vi "Numerique_vers_chaine.vi"(0 "Valeur numérique":dbl) -> (1 "Chaine sans zéros inutiles":string, 2 "Chaîne brute":string)   [LabVIEW 2022 SP3]
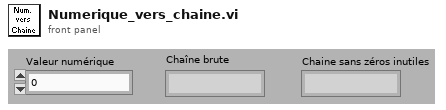
[diagram p1: front panel]
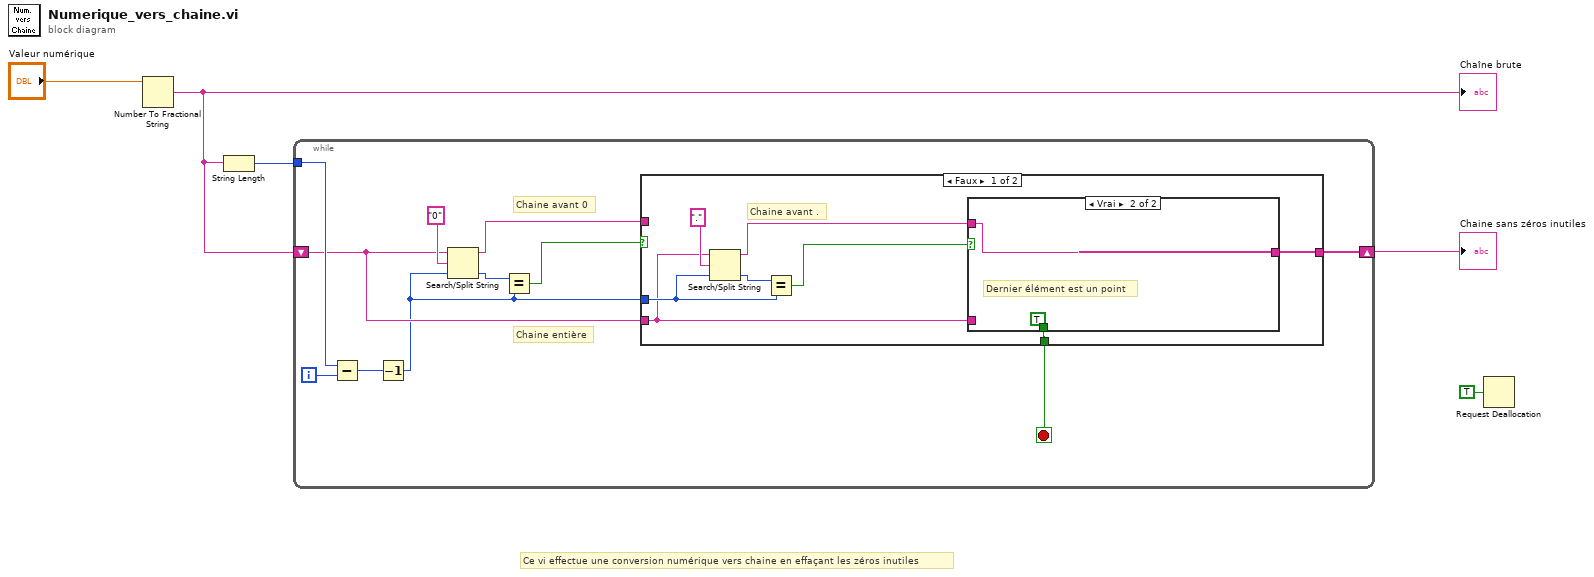
[diagram p0: block diagram]
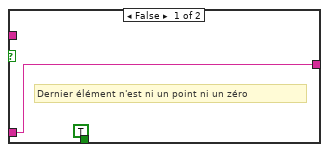
[diagram p2: hidden frame]
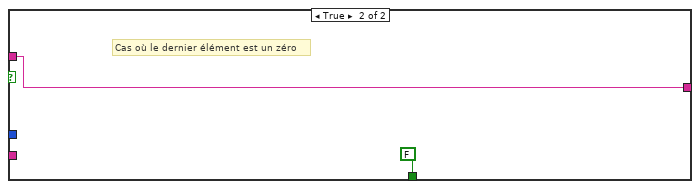
[diagram p3: hidden frame]
diagram:
  # "Ce vi effectue une conversion numérique vers chaine en effaçant les zéros inutiles"
  n1 = Number To Fractional String(number="Valeur numérique") -> (F-format string=w2:string)  [unwired: 3 in]
  "Chaîne brute" <- w2
  n2 = String Length(string=w2) -> (length=w4:i32)
  n3 = while {
    shift-right: [w9] -> w3
    shift-left: w2 -> [w8]
    tunnel: w4 -> [w10]
    i -> [w11]
    stop <- w6 stop-if-true
    # "Chaine entière"
    # "Chaine avant 0"
    n4 = Subtract(x=w10, y=w11) -> (x-y=w16:i32)
    n5 = Decrement(x=w16) -> (x-1=w7:i32)
    n6 = Search/Split String(string=w8, search string/char (-)="0" ("chaîne/car. recherché (-)"), offset (0)=w7) -> (substring before match=w12:string, offset of match=w14:i32)  [unwired: 1 out]
    n7 = Equal?(x=w14, y=w7) -> (x = y?=w13:bool)
    n8 = case shown="Faux" w13 {
      tunnel: w12 -> [_ w30]
      tunnel: [w18 w30] -> w9
      tunnel: w8 -> [w17 _]
      tunnel: w7 -> [w20 _]
      tunnel: [w19 FALSE] -> w6
      frame False {
        # "Chaine avant ."
        n9 = Search/Split String(string=w17, search string/char (-)="." ("chaîne/car. recherché (-)"), offset (0)=w20) -> (substring before match=w22:string, offset of match=w24:i32)  [unwired: 1 out]
        n10 = Equal?(x=w24, y=w20) -> (x = y?=w21:bool)
        n11 = case shown="Vrai" w21 {
          tunnel: w22 -> [_ w28]
          tunnel: [w25 w28] -> w18
          tunnel: [TRUE TRUE] -> w19
          tunnel: w17 -> [w25 _]
          frame False {
            # "Dernier élément n'est ni un point ni un zéro"
          }
          frame True {
            # "Dernier élément est un point"
          }
        }
      }
      frame True {
        # "Cas où le dernier élément est un zéro"
      }
    }
  }
  "Chaine sans zéros inutiles" <- w3
  n12 = Request Deallocation(TRUE ("flag")) -> ()
